vi "Acquistions.vi"() -> ()   [LabVIEW 2022 SP3]
uses:
  Enum/Enum p2.ctl
  Variables globales/Variable glob Leybold.vi
  Variables globales/Variable glob Edwards.vi
  Variables globales/Variable glob Keller.vi
  Variables globales/Variable glob Th.vi
  Variables globales/Variable glob Pt.vi
  Variables globales/Variables glob EUROTHERM.vi
  Variables globales/Variable globale compteurs.vi
panel:
  out "ref compteur":refnum<vi>
  out "ref EDWARDS grappes":refnum<vi>
  out "ref Reg":refnum<vi>
  out "ref Pt":refnum<vi>
  out "ref Th":refnum<vi>
  out "ref KELLER":refnum<vi>
  out "ref EDWARDS":refnum<vi>
  out "ref LEYBOLD":refnum<vi>
  in  "Chaîne":string="\nAcquisitions\nen cours de\nlancement"
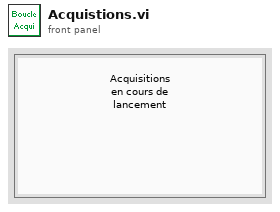
[diagram p1: front panel]
types:
  T1 = typedef "Enum p2.ctl" = enum16{"Init", "LEYBOLD", "EDWARDS", "KELLER", "Th", "Pt", "REG", "COMPTEURS", "fin"}
  T2 = enum32{"Bad", "Idle", "Run top level", "Running"}
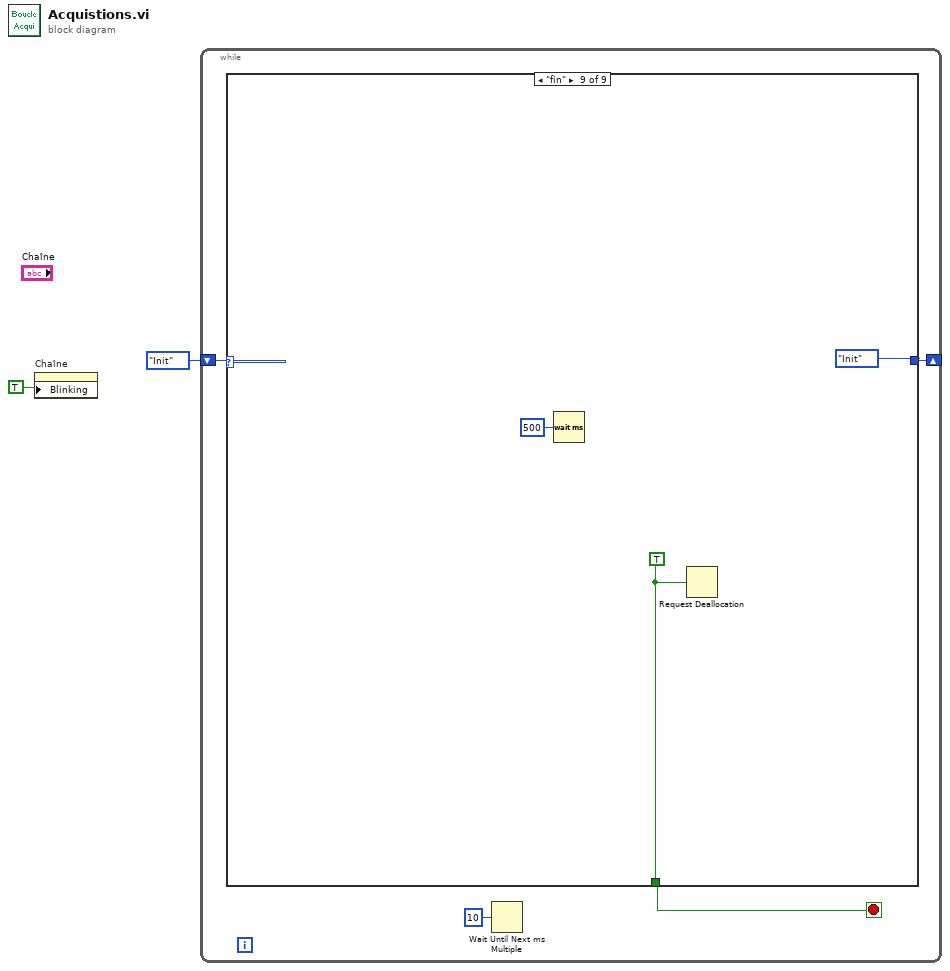
[diagram p0: block diagram]
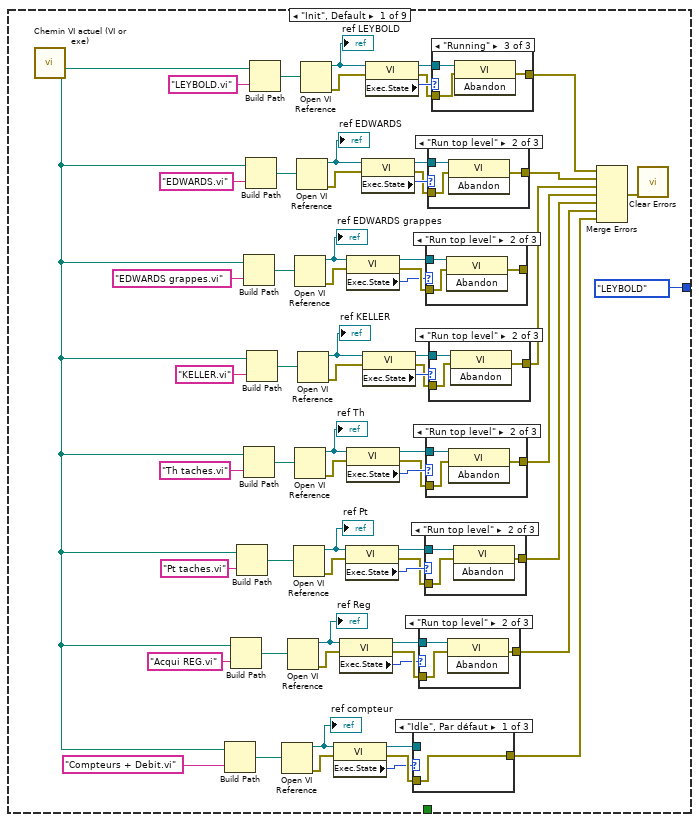
[diagram p2: hidden frame]
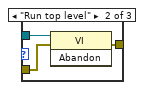
[diagram p3: hidden frame]
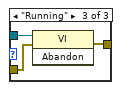
[diagram p4: hidden frame]
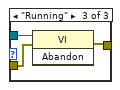
[diagram p6: hidden frame]
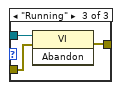
[diagram p8: hidden frame]
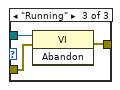
[diagram p10: hidden frame]
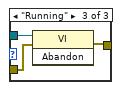
[diagram p12: hidden frame]
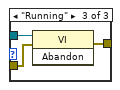
[diagram p14: hidden frame]
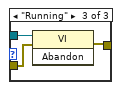
[diagram p16: hidden frame]
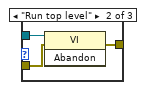
[diagram p18: hidden frame]
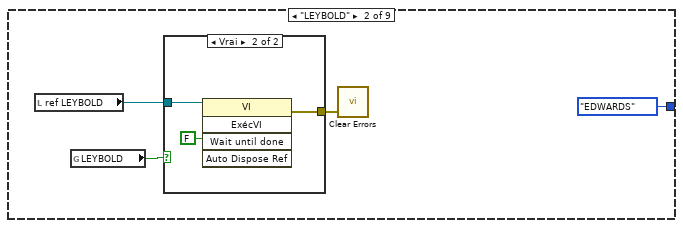
[diagram p19: hidden frame]
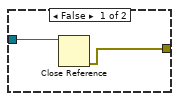
[diagram p20: hidden frame]
diagram:
  n1 = property on="Chaîne" class="Ch"("Blinking"=TRUE) -> ()  [unwired: 2 in, 2 out]
  n2 = while {
    shift-right: [w4] -> _
    shift-left: Enum_p2."Init" ("Énum") -> [w6]
    stop <- w5 stop-if-true
    n3 = case shown="\"fin\"" w6 {
      tunnel: [_ _ _ _ _ _ _ _ w201] -> w5
      tunnel: [Enum_p2."LEYBOLD" ("Énum") Enum_p2."EDWARDS" ("Énum") Enum_p2."KELLER" ("Énum") Enum_p2."Th" ("Énum") Enum_p2."Pt" ("Énum") Enum_p2."REG" ("Énum") Enum_p2."COMPTEURS" ("Énum") Enum_p2."fin" ("Énum") Enum_p2."Init" ("Énum")] -> w4
      frame "Init", Default {
        n4 = call "Chemin VI actuel (VI or exe).vi"() -> ("VI or executable installation directory"=w8:path)  [unwired: 14 in, 1 out]
        n5 = Build Path(base path=w8, name or relative path="Compteurs + Debit.vi" ("nom ou chemin relatif")) -> (appended path=w10:path)
        n6 = Build Path(base path=w8, name or relative path="Acqui REG.vi" ("nom ou chemin relatif")) -> (appended path=w25:path)
        n7 = Build Path(base path=w8, name or relative path="Pt taches.vi" ("nom ou chemin relatif")) -> (appended path=w50:path)
        n8 = Build Path(base path=w8, name or relative path="EDWARDS grappes.vi" ("nom ou chemin relatif")) -> (appended path=w19:path)
        n9 = Build Path(base path=w8, name or relative path="Th taches.vi" ("nom ou chemin relatif")) -> (appended path=w53:path)
        n10 = Build Path(base path=w8, name or relative path="EDWARDS.vi" ("nom ou chemin relatif")) -> (appended path=w63:path)
        n11 = Build Path(base path=w8, name or relative path="KELLER.vi" ("nom ou chemin relatif")) -> (appended path=w60:path)
        n12 = Build Path(base path=w8, name or relative path="LEYBOLD.vi" ("nom ou chemin relatif")) -> (appended path=w70:path)
        n13 = Open VI Reference(vi path=w10) -> (vi reference=w15:refnum<vi>, error out=w14:errorcluster)  [unwired: 5 in]
        "ref compteur" <- w15
        n14 = Open VI Reference(vi path=w25) -> (vi reference=w30:refnum<vi>, error out=w29:errorcluster)  [unwired: 5 in]
        "ref Reg" <- w30
        n15 = Open VI Reference(vi path=w50) -> (vi reference=w37:refnum<vi>, error out=w42:errorcluster)  [unwired: 5 in]
        "ref Pt" <- w37
        n16 = Open VI Reference(vi path=w19) -> (vi reference=w18:refnum<vi>, error out=w22:errorcluster)  [unwired: 5 in]
        "ref EDWARDS grappes" <- w18
        n17 = Open VI Reference(vi path=w53) -> (vi reference=w54:refnum<vi>, error out=w41:errorcluster)  [unwired: 5 in]
        "ref Th" <- w54
        n18 = Open VI Reference(vi path=w63) -> (vi reference=w64:refnum<vi>, error out=w39:errorcluster)  [unwired: 5 in]
        "ref EDWARDS" <- w64
        n19 = Open VI Reference(vi path=w60) -> (vi reference=w59:refnum<vi>, error out=w40:errorcluster)  [unwired: 5 in]
        "ref KELLER" <- w59
        n20 = Open VI Reference(vi path=w70) -> (vi reference=w69:refnum<vi>, error out=w38:errorcluster)  [unwired: 5 in]
        "ref LEYBOLD" <- w69
        n21 = property class="VI"(reference=w15, error in=w14) -> (reference out=w12:refnum<vi>, error out=w13:errorcluster, "Exec.State"=w11:T2)
        n22 = property class="VI"(reference=w30, error in=w29) -> (reference out=w27:refnum<vi>, error out=w28:errorcluster, "Exec.State"=w26:T2)
        n23 = property class="VI"(reference=w37, error in=w42) -> (reference out=w48:refnum<vi>, error out=w43:errorcluster, "Exec.State"=w49:T2)
        n24 = property class="VI"(reference=w18, error in=w22) -> (reference out=w16:refnum<vi>, error out=w21:errorcluster, "Exec.State"=w17:T2)
        n25 = property class="VI"(reference=w54, error in=w41) -> (reference out=w56:refnum<vi>, error out=w44:errorcluster, "Exec.State"=w55:T2)
        n26 = property class="VI"(reference=w64, error in=w39) -> (reference out=w66:refnum<vi>, error out=w46:errorcluster, "Exec.State"=w65:T2)
        n27 = property class="VI"(reference=w59, error in=w40) -> (reference out=w57:refnum<vi>, error out=w45:errorcluster, "Exec.State"=w58:T2)
        n28 = property class="VI"(reference=w69, error in=w38) -> (reference out=w67:refnum<vi>, error out=w47:errorcluster, "Exec.State"=w68:T2)
        n29 = case shown="\"Idle\", Par défaut" w11 {
          tunnel: w12 -> [_ w76 w79]
          tunnel: w13 -> [w73 w75 w78]
          tunnel: [w73 w74 w77] -> w7
          frame "Idle", Default {
          }
          frame "Run top level" {
            n30 = invoke class="VI" method="Abandon"(reference=w76, error in=w75) -> (error out=w74:errorcluster)  [unwired: 1 in, 2 out]
          }
          frame "Running" {
            n31 = invoke class="VI" method="Abandon"(reference=w79, error in=w78) -> (error out=w77:errorcluster)  [unwired: 1 in, 2 out]
          }
        }
        n32 = case shown="\"Run top level\"" w26 {
          tunnel: w27 -> [_ w90 w93]
          tunnel: w28 -> [w87 w89 w92]
          tunnel: [w87 w88 w91] -> w23
          frame "Idle", Default {
          }
          frame "Run top level" {
            n33 = invoke class="VI" method="Abandon"(reference=w90, error in=w89) -> (error out=w88:errorcluster)  [unwired: 1 in, 2 out]
          }
          frame "Running" {
            n34 = invoke class="VI" method="Abandon"(reference=w93, error in=w92) -> (error out=w91:errorcluster)  [unwired: 1 in, 2 out]
          }
        }
        n35 = case shown="\"Run top level\"" w49 {
          tunnel: w48 -> [_ w97 w100]
          tunnel: w43 -> [w94 w96 w99]
          tunnel: [w94 w95 w98] -> w34
          frame "Idle", Default {
          }
          frame "Run top level" {
            n36 = invoke class="VI" method="Abandon"(reference=w97, error in=w96) -> (error out=w95:errorcluster)  [unwired: 1 in, 2 out]
          }
          frame "Running" {
            n37 = invoke class="VI" method="Abandon"(reference=w100, error in=w99) -> (error out=w98:errorcluster)  [unwired: 1 in, 2 out]
          }
        }
        n38 = case shown="\"Run top level\"" w17 {
          tunnel: w16 -> [_ w83 w86]
          tunnel: w21 -> [w80 w82 w85]
          tunnel: [w80 w81 w84] -> _
          frame "Idle", Default {
          }
          frame "Run top level" {
            n39 = invoke class="VI" method="Abandon"(reference=w83, error in=w82) -> (error out=w81:errorcluster)  [unwired: 1 in, 2 out]
          }
          frame "Running" {
            n40 = invoke class="VI" method="Abandon"(reference=w86, error in=w85) -> (error out=w84:errorcluster)  [unwired: 1 in, 2 out]
          }
        }
        n41 = case shown="\"Run top level\"" w55 {
          tunnel: w56 -> [_ w104 w107]
          tunnel: w44 -> [w101 w103 w106]
          tunnel: [w101 w102 w105] -> w33
          frame "Idle", Default {
          }
          frame "Run top level" {
            n42 = invoke class="VI" method="Abandon"(reference=w104, error in=w103) -> (error out=w102:errorcluster)  [unwired: 1 in, 2 out]
          }
          frame "Running" {
            n43 = invoke class="VI" method="Abandon"(reference=w107, error in=w106) -> (error out=w105:errorcluster)  [unwired: 1 in, 2 out]
          }
        }
        n44 = case shown="\"Run top level\"" w65 {
          tunnel: w66 -> [_ w118 w121]
          tunnel: w46 -> [w115 w117 w120]
          tunnel: [w115 w116 w119] -> w35
          frame "Idle", Default {
          }
          frame "Run top level" {
            n45 = invoke class="VI" method="Abandon"(reference=w118, error in=w117) -> (error out=w116:errorcluster)  [unwired: 1 in, 2 out]
          }
          frame "Running" {
            n46 = invoke class="VI" method="Abandon"(reference=w121, error in=w120) -> (error out=w119:errorcluster)  [unwired: 1 in, 2 out]
          }
        }
        n47 = case shown="\"Run top level\"" w58 {
          tunnel: w57 -> [_ w111 w114]
          tunnel: w45 -> [w108 w110 w113]
          tunnel: [w108 w109 w112] -> w32
          frame "Idle", Default {
          }
          frame "Run top level" {
            n48 = invoke class="VI" method="Abandon"(reference=w111, error in=w110) -> (error out=w109:errorcluster)  [unwired: 1 in, 2 out]
          }
          frame "Running" {
            n49 = invoke class="VI" method="Abandon"(reference=w114, error in=w113) -> (error out=w112:errorcluster)  [unwired: 1 in, 2 out]
          }
        }
        n50 = case shown="\"Running\"" w68 {
          tunnel: w67 -> [_ w125 w128]
          tunnel: w47 -> [w122 w124 w127]
          tunnel: [w122 w123 w126] -> w36
          frame "Idle", Default {
          }
          frame "Run top level" {
            n51 = invoke class="VI" method="Abandon"(reference=w125, error in=w124) -> (error out=w123:errorcluster)  [unwired: 1 in, 2 out]
          }
          frame "Running" {
            n52 = invoke class="VI" method="Abandon"(reference=w128, error in=w127) -> (error out=w126:errorcluster)  [unwired: 1 in, 2 out]
          }
        }
        n53 = Merge Errors(w36, w35, w32, w33, w34, w23, w7) -> (w31:errorcluster)
        n54 = call <vilib>:"Clear Errors.vi"("error in (no error)"=w31) -> ()  [unwired: 5 in, 2 out]
      }
      frame "LEYBOLD" {
        n55 = local read "ref LEYBOLD"() -> (w130:refnum<vi>)
        n56 = global read "Variable glob Leybold.vi" "LEYBOLD"() -> (w131:bool)
        n57 = case shown="Vrai" w131 {
          tunnel: w130 -> [w134 w136]
          tunnel: [w133 w135] -> w129
          frame False {
            n58 = Close Reference(reference=w134) -> (error out=w133:errorcluster)  [unwired: 1 in]
          }
          frame True {
            n59 = invoke class="VI" method="ExécVI"(reference=w136, "Wait until done"=FALSE ("Attendre la fin")) -> (error out=w135:errorcluster)  [unwired: 3 in, 4 out]
          }
        }
        n60 = call <vilib>:"Clear Errors.vi"("error in (no error)"=w129) -> ()  [unwired: 5 in, 2 out]
      }
      frame "EDWARDS" {
        n61 = local read "ref EDWARDS grappes"() -> (w138:refnum<vi>)
        n62 = local read "ref EDWARDS"() -> (w141:refnum<vi>)
        n63 = global read "Variable glob Edwards.vi" "EDWARDS"() -> (w140:bool)
        n64 = case shown="Vrai" w140 {
          tunnel: w141 -> [w147 w153]
          tunnel: [w143 w148] -> w139
          tunnel: w138 -> [w146 w151]
          frame False {
            n65 = Close Reference(reference=w146) -> (error out=w144:errorcluster)  [unwired: 1 in]
            n66 = Close Reference(reference=w147) -> (error out=w145:errorcluster)  [unwired: 1 in]
            n67 = Merge Errors(w145, w144) -> (w143:errorcluster)
          }
          frame True {
            n68 = invoke class="VI" method="ExécVI"(reference=w153, "Wait until done"=FALSE ("Attendre la fin")) -> (error out=w150:errorcluster)  [unwired: 3 in, 4 out]
            n69 = invoke class="VI" method="ExécVI"(reference=w151, "Wait until done"=FALSE ("Attendre la fin")) -> (error out=w149:errorcluster)  [unwired: 3 in, 4 out]
            n70 = Merge Errors(w150, w149) -> (w148:errorcluster)
          }
        }
        n71 = call <vilib>:"Clear Errors.vi"("error in (no error)"=w139) -> ()  [unwired: 5 in, 2 out]
      }
      frame "KELLER" {
        n72 = local read "ref KELLER"() -> (w157:refnum<vi>)
        n73 = global read "Variable glob Keller.vi" "KELLER"() -> (w156:bool)
        n74 = case shown="Faux" w156 {
          tunnel: w157 -> [w160 w162]
          tunnel: [w159 w161] -> w155
          frame False {
            n75 = Close Reference(reference=w160) -> (error out=w159:errorcluster)  [unwired: 1 in]
          }
          frame True {
            n76 = invoke class="VI" method="ExécVI"(reference=w162, "Wait until done"=FALSE ("Attendre la fin")) -> (error out=w161:errorcluster)  [unwired: 3 in, 4 out]
          }
        }
        n77 = call <vilib>:"Clear Errors.vi"("error in (no error)"=w155) -> ()  [unwired: 5 in, 2 out]
      }
      frame "Th" {
        n78 = global read "Variable glob Th.vi" "Temp Th"() -> (w165:bool)
        n79 = local read "ref Th"() -> (w166:refnum<vi>)
        n80 = case shown="Faux" w165 {
          tunnel: w166 -> [w169 w171]
          tunnel: [w168 w170] -> w164
          frame False {
            n81 = Close Reference(reference=w169) -> (error out=w168:errorcluster)  [unwired: 1 in]
          }
          frame True {
            n82 = invoke class="VI" method="ExécVI"(reference=w171, "Wait until done"=FALSE ("Attendre la fin")) -> (error out=w170:errorcluster)  [unwired: 3 in, 4 out]
          }
        }
        n83 = call <vilib>:"Clear Errors.vi"("error in (no error)"=w164) -> ()  [unwired: 5 in, 2 out]
      }
      frame "Pt" {
        n84 = global read "Variable glob Pt.vi" "Temp Pt"() -> (w175:bool)
        n85 = local read "ref Pt"() -> (w174:refnum<vi>)
        n86 = case shown="Vrai" w175 {
          tunnel: w174 -> [w178 w180]
          tunnel: [w177 w179] -> w173
          frame False {
            n87 = Close Reference(reference=w178) -> (error out=w177:errorcluster)  [unwired: 1 in]
          }
          frame True {
            n88 = invoke class="VI" method="ExécVI"(reference=w180, "Wait until done"=FALSE ("Attendre la fin")) -> (error out=w179:errorcluster)  [unwired: 3 in, 4 out]
          }
        }
        n89 = call <vilib>:"Clear Errors.vi"("error in (no error)"=w173) -> ()  [unwired: 5 in, 2 out]
      }
      frame "REG" {
        n90 = local read "ref Reg"() -> (w182:refnum<vi>)
        n91 = global read "Variables glob EUROTHERM.vi" "REG"() -> (w183:bool)
        n92 = case shown="Vrai" w183 {
          tunnel: w182 -> [w187 w189]
          tunnel: [w186 w188] -> w184
          frame False {
            n93 = Close Reference(reference=w187) -> (error out=w186:errorcluster)  [unwired: 1 in]
          }
          frame True {
            n94 = invoke class="VI" method="ExécVI"(reference=w189, "Wait until done"=FALSE ("Attendre la fin")) -> (error out=w188:errorcluster)  [unwired: 3 in, 4 out]
          }
        }
        n95 = call <vilib>:"Clear Errors.vi"("error in (no error)"=w184) -> ()  [unwired: 5 in, 2 out]
      }
      frame "COMPTEURS" {
        n96 = local read "ref compteur"() -> (w192:refnum<vi>)
        n97 = global read "Variable globale compteurs.vi" "COMPTEURS"() -> (w191:bool)
        n98 = case shown="Vrai" w191 {
          tunnel: w192 -> [w196 w198]
          tunnel: [w195 w197] -> w193
          frame False {
            n99 = Close Reference(reference=w196) -> (error out=w195:errorcluster)  [unwired: 1 in]
          }
          frame True {
            n100 = invoke class="VI" method="ExécVI"(reference=w198, "Wait until done"=FALSE ("Attendre la fin")) -> (error out=w197:errorcluster)  [unwired: 3 in, 4 out]
          }
        }
        n101 = call <vilib>:"Clear Errors.vi"("error in (no error)"=w193) -> ()  [unwired: 5 in, 2 out]
      }
      frame "fin" {
        w201 = TRUE
        n102 = Wait (ms)(milliseconds to wait=u32 500 ("attente (ms)")) -> ()  [unwired: 1 out]
        n103 = Request Deallocation(w201) -> ()
      }
    }
    n104 = Wait Until Next ms Multiple(millisecond multiple=u32 10 ("n millisecondes")) -> ()  [unwired: 1 out]
  }
